vi "Read String Direct.vi"(8 "error in (no error)":errorcluster, 11 "CIFTag in":refnum<class "CIF_Iceoryx_Chn_String.lvclass">) -> (0 "error out":errorcluster, 2 "Data":string, 3 "CIFTag out":refnum<class "CIF_Iceoryx_Chn_String.lvclass">)   [LabVIEW 2021, in "CIF_Iceoryx_Chn_String.lvclass"]
uses:
  CIF_Iceoryx_Chn_String.lvclass
  D:/dev/Packages/CIF_Channels_Core/src/CIFChannels/CIFChannels.lvclass
  D:/dev/Packages/CIF_Channels_Core/src/Iceorxy_Channels/CIF_Iceoryx_BB/CIF_Iceoryx_BB.lvclass
  CIFChannels/CIFChannels.lvclass/CIFChannels.ctl
  ChannelCommon/typedef/Channel State.ctl
  ChannelCommon/typedef/Direction.ctl
  CIF_Iceoryx_Chn_String.lvclass/CIF_Iceoryx_Chn_String.ctl
  CIF_Iceoryx_BB/CIF_Iceoryx_BB.lvclass/CIF_Iceoryx_BB.ctl
  CIFChannels/Accessors/Read Channel State.vi
  CIFChannels/Accessors/Read Direction.vi
  CIFChannels/Accessors/Read Tag Forced.vi
  <vilib>/CIF Foundation/CIF Iceoryx/SubVIs/Get Path.vi
  <vilib>/CIF Foundation/CIF Iceoryx/SubVIs/Convert Error.vi
  <vilib>/CIF Foundation/CIF Iceoryx/Refnum/BB Reader from Refnum.vi
  <vilib>/CIF Foundation/CIF Iceoryx/SubVIs/Convert Error Core.vi
  ChannelCommon/ChannelCommon.lvlib
  f7b43f44-818d-49c1-b9e3-1feecbab48db.vi
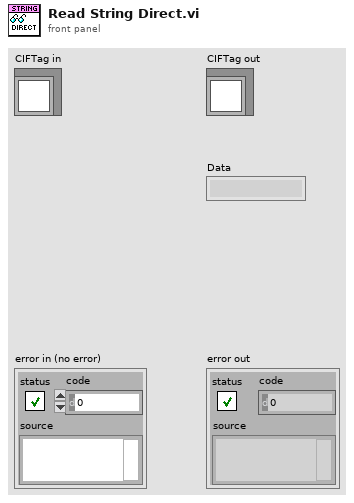
[diagram p1: front panel]
types:
  T1 = typedef "ChannelCommon.lvlib/Channel State.ctl" = enum8{"Creating", "Disconnected", "Connecting", "Connected", "Destroyed"}
  T2 = typedef "ChannelCommon.lvlib/Direction.ctl" = enum8{"Publisher", "Subscriber"}
  T3 = typedef "Iceoryx.lvlib/BB Reader Refnum.ctl" = cluster{"refnum":u64, "BB Reader":enum8{"bb_reader"}}
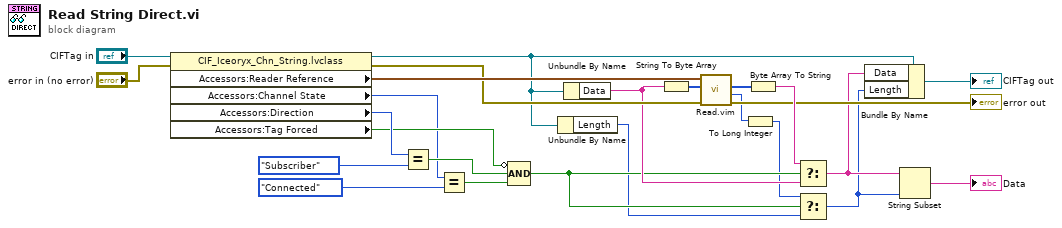
[diagram p0: block diagram]
diagram:
  n1 = property class="CIF_Iceoryx_Chn_String.lvclass"(reference="CIFTag in", error in="error in (no error)") -> (reference out=w7:refnum<class "CIF_Iceoryx_Chn_String.lvclass">, error out=w17:errorcluster, "Accessors:Reader Reference"=w18:T3, "Accessors:Channel State"=w19:T1, "Accessors:Direction"=w25:T2, "Accessors:Tag Forced"=w20:bool)
  n2 = Equal?(x=w25, y=Direction."Subscriber") -> (x = y?=w21:bool)
  n3 = Equal?(x=w19, y=Channel_State."Connected") -> (x = y?=w22:bool)
  n4 = Compound Arithmetic op=AND(invert w20, w21, w22) -> (w8:bool)
  n5 = Unbundle By Name(w7) -> ("Length"=w6:i32)
  n6 = Unbundle By Name(w7) -> ("Data"=w11:string)
  n7 = String To Byte Array(string=w11) -> (unsigned byte array=w14:u8[])
  n8 = call "Read.vim"("error in (no error)"=w17, "Data In"=w14, "Reader Reference"=w18) -> ("error out"=→"error out":errorcluster, "Array Length"=w5:u32, "Data Out"=w13:u8[])  [unwired: 6 in]
  n9 = To Long Integer(number=w5) -> (32bit integer=w4:i32)
  n10 = Byte Array To String(unsigned byte array=w13) -> (string=w12:string)
  n11 = Select(t=w12, s=w8, f=w11) -> (s? t:f=w3:string)
  n12 = Select(t=w4, s=w8, f=w6) -> (s? t:f=w1:i32)
  n13 = Bundle By Name(cluster=w7, "Data"=w3, "Length"=w1) -> (→"CIFTag out":refnum<class "CIF_Iceoryx_Chn_String.lvclass">)
  n14 = String Subset(string=w3, length (rest)=w1) -> (substring=→"Data":string)  [unwired: 1 in]
